vi "Timer_Example_1.vi"() -> ()   [LabVIEW 2019]
uses:
  <vilib>/Utility/semaphor.llb/Obtain Semaphore Reference.vi
  <vilib>/Rock Robotics/WPI/ThirdParty/JAS_Junk/TrajLib/Trajectory_Library.lvlib
panel:
  in  "Tab Control":enum32{"Control Panel"}(tab)
  in  "Restart Timer":bool
  in  "Reset TImer":bool
  in  "Stop Timer":bool
  in  "Start Timer":bool
  out "Trend":cluster{"CurrentTImer":dbl, "CurrentTImer":dbl}(graph)
  out "Expired":bool
  out "Timer 2":dbl
  out "Timer 1":dbl
  # "Timer Example 1"
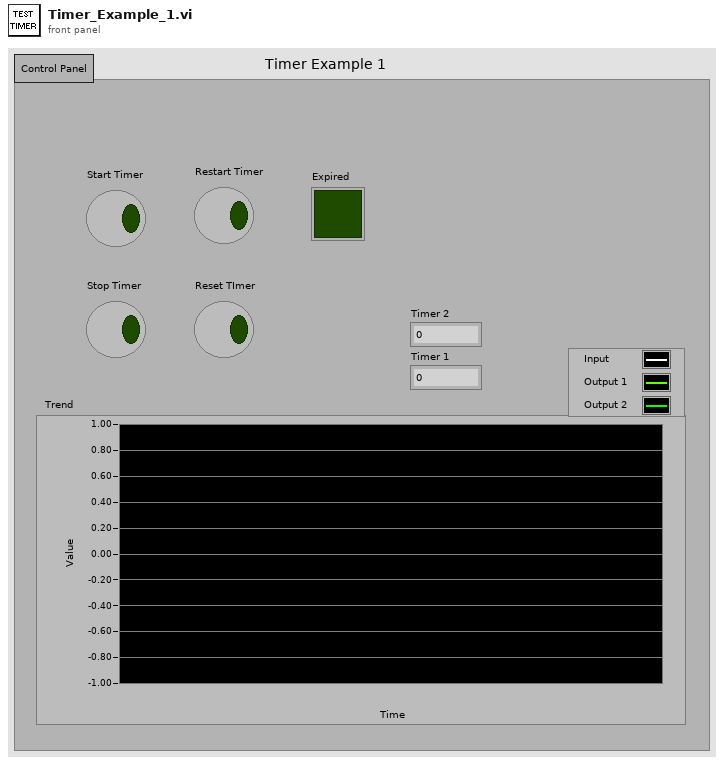
[diagram p1: front panel]
types:
  T1 = typedef "Trajectory_Library.lvlib/TIMER.ctl" = cluster{"StartTime":dbl, "Accumulated TIme":dbl, "Running":bool, "semaphore":T2}
  T2 = typedef "Semaphore RefNum" = refnum<k1>
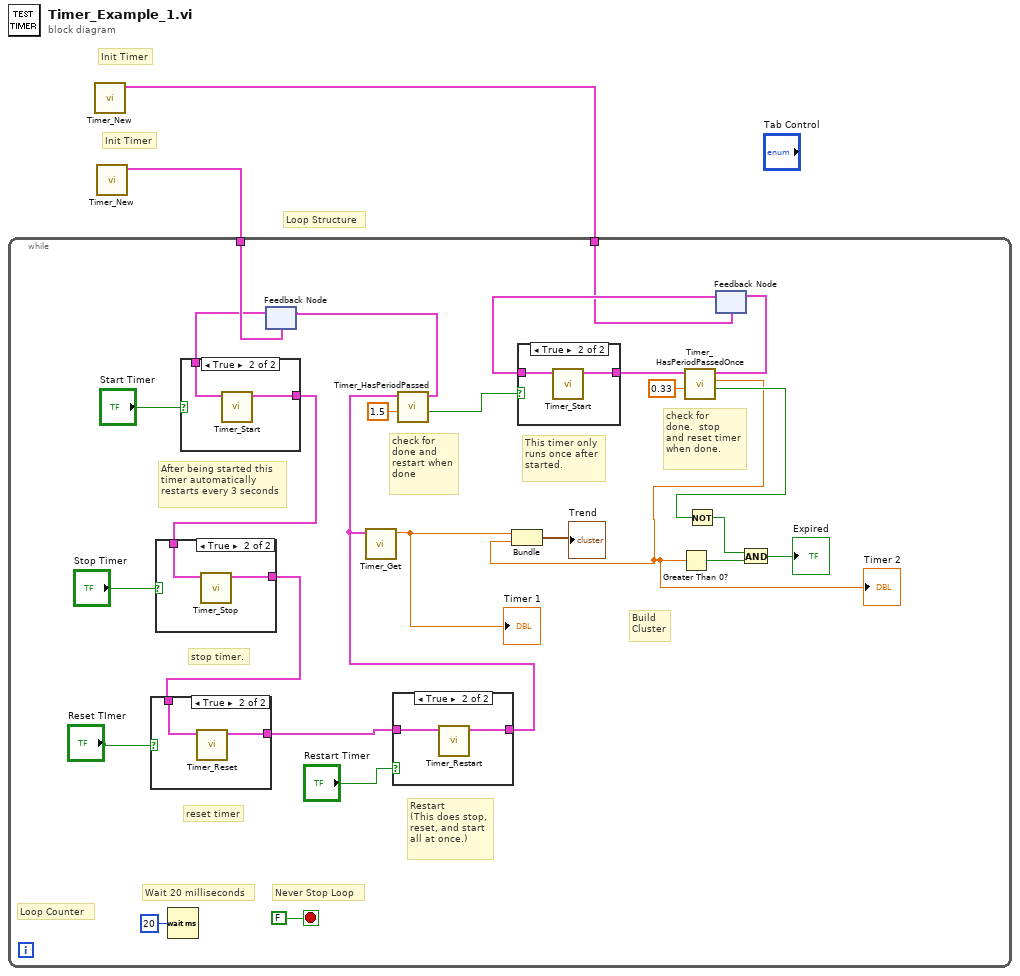
[diagram p0: block diagram]
diagram:
  # "Init Timer"
  # "Init Timer"
  # "Loop Structure"
  n1 = call <vilib>:"Timer_New.vi"() -> ("TIMER"=w1:T1)  [unwired: 11 in]
  n2 = call <vilib>:"Timer_New.vi"() -> ("TIMER"=w2:T1)  [unwired: 11 in]
  n3 = while {
    tunnel: w2 -> [w26]
    tunnel: w1 -> [w21]
    stop <- FALSE stop-if-true
    # "Restart\n(This does stop,\nreset, and start\nall at once.)"
    # "reset timer"
    # "stop timer."
    # "This timer only\nruns once after\nstarted."
    # "check for\ndone.  stop\nand reset timer\nwhen done."
    # "check for\ndone and\nrestart when\ndone"
    # "After being started this \ntimer automatically\nrestarts every 3 seconds"
    # "Build\nCluster"
    # "Loop Counter"
    # "Never Stop Loop"
    # "Wait 20 milliseconds"
    n4 = Wait (ms)(milliseconds to wait=u32 20) -> ()  [unwired: 1 out]
    n5 = feedback #1(w26) -> (w25:T1)
    n6 = case shown="True" "Start Timer" {
      tunnel: [w42 w44] -> w8
      tunnel: w25 -> [w42 w43]
      frame False {
      }
      frame True {
        n7 = call <vilib>:"Timer_Start.vi"("in Timer"=w43) -> ("out Timer"=w44:T1)  [unwired: 10 in]
      }
    }
    n8 = case shown="True" "Stop Timer" {
      tunnel: [w36 w38] -> w6
      tunnel: w8 -> [w36 w37]
      frame False {
      }
      frame True {
        n9 = call <vilib>:"Timer_Stop.vi"("in Timer"=w37) -> ("out Timer"=w38:T1)  [unwired: 10 in]
      }
    }
    n10 = case shown="True" "Reset TImer" {
      tunnel: [w33 w34] -> w5
      tunnel: w6 -> [w33 w35]
      frame False {
      }
      frame True {
        n11 = call <vilib>:"Timer_Reset.vi"("in TIMER"=w35) -> ("out TIMER"=w34:T1)  [unwired: 10 in]
      }
    }
    n12 = case shown="True" "Restart Timer" {
      tunnel: [w30 w32] -> w3
      tunnel: w5 -> [w30 w31]
      frame False {
      }
      frame True {
        n13 = call <vilib>:"Timer_Restart.vi"("in Timer"=w31) -> ("out Timer"=w32:T1)  [unwired: 10 in]
      }
    }
    n14 = call <vilib>:"Timer_Get.vi"("TIMER"=w3) -> ("CurrentTImer"=w13:dbl)  [unwired: 10 in]
    "Timer 1" <- w13
    n15 = call <vilib>:"Timer_HasPeriodPassed.vi"("Period"=1.5, "in Timer"=w3) -> ("Expired"=w19:bool, "out Timer"=w24:T1)  [unwired: 7 in, 1 out]
    n16 = feedback-in #1(w24) -> ()
    n17 = feedback #2(w21) -> (w22:T1)
    n18 = case shown="True" w19 {
      tunnel: w22 -> [w39 w41]
      tunnel: [w39 w40] -> w14
      frame False {
      }
      frame True {
        n19 = call <vilib>:"Timer_Start.vi"("in Timer"=w41) -> ("out Timer"=w40:T1)  [unwired: 10 in]
      }
    }
    n20 = call <vilib>:"Timer_HasPeriodPassedOnce.vi"("Period"=0.33, "in Timer"=w14) -> ("Expired"=w18:bool, "CurrentTImer"=w10:dbl, "out Timer"=w11:T1)  [unwired: 7 in]
    "Timer 2" <- w10
    n21 = Bundle("CurrentTImer"=w13, "CurrentTImer"=w10) -> (→"Trend":cluster{"CurrentTImer":dbl, "CurrentTImer":dbl})  [unwired: 1 in]
    n22 = Greater Than 0?(x=w10) -> (x > 0?=w15:bool)
    n23 = Not(x=w18) -> (.not. x?=w16:bool)
    n24 = feedback-in #2(w11) -> ()
    n25 = And(x=w16, y=w15) -> (x .and. y?=→"Expired":bool)
  }
